vi "MQTT Data - Encode String.vi"(7 "String in":string, 9 "To UTF-8?":bool=TRUE, 11 "error in (no error)":errorcluster) -> (8 "Bytes out":u8[](array[numeric]), 15 "error out":errorcluster)   [LabVIEW 2019, in "KoRE-MQTT.lvlib"]
doc: "Copyright (c) 2025 KoRElibs.com\nSPDX-License-Identifier: EUPL-1.2\n\nThis VI is licensed under the European Union Public License (EUPL) Version 1.2. You may use this VI unmodified in proprietary works. If you distribute a modified version of this file, the modified file must be released under the EUPL-1.2. Full license: https://joinup.ec.europa.eu/asset/eupl/eupl/1.2/"
uses:
  KoRE-MQTT.lvlib
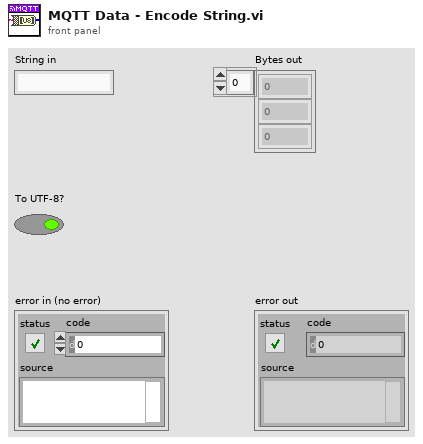
[diagram p1: front panel]
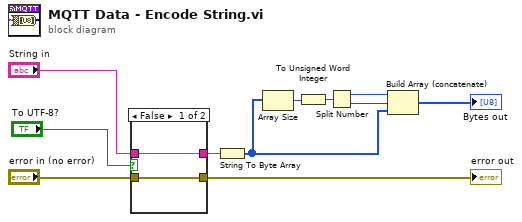
[diagram p0: block diagram]
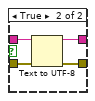
[diagram p2: hidden frame]
diagram:
  n1 = case shown="False" "To UTF-8?" {
    tunnel: "String in" -> [w13 w17]
    tunnel: "error in (no error)" -> [w12 w16]
    tunnel: [w13 w15] -> w9
    tunnel: [w12 w14] -> w2
    frame False {
    }
    frame True {
      n2 = Text to UTF-8(8:w16, 11:w17) -> (0:w14:errorcluster, 3:w15:string)  [unwired: 1 in]
    }
  }
  "error out" <- w2
  n3 = String To Byte Array(string=w9) -> (unsigned byte array=w8:u8[])
  n4 = Array Size(array=w8) -> (size(s)=w7:i32)
  n5 = To Unsigned Word Integer(number=w7) -> (unsigned 16bit integer=w3:u16)
  n6 = Split Number(x=w3) -> (hi(x)=w5:u8, lo(x)=w6:u8)
  n7 = Build Array (concatenate)(w5, w6, w8) -> (→"Bytes out":u8[])
